vi "Remove Task.vi"(7 "Project Store in":refnum<class "Project Store.lvclass">, 8 "error in (no error)":errorcluster, 11 "ID":string) -> (0 "error out":errorcluster, 3 "found?":bool, 5 "Project Store out":refnum<class "Project Store.lvclass">)   [LabVIEW 2024, in "Project Store.lvclass"]
doc: "Removes the task with the given ID from the in-memory model. found? is FALSE when no task has that ID. Nothing is written to disk until Write to Data Source.\n\nGenerated by: Claude"
uses:
  Project Store.lvclass
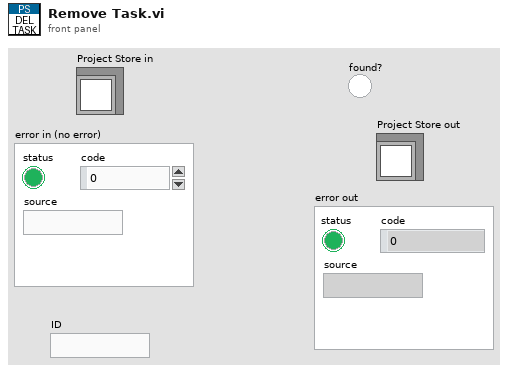
[diagram p1: front panel]
types:
  T1 = typedef "Task List.ctl" = T2[]
  T2 = typedef "Task.ctl" = cluster{"ID":string, "Project ID":string, "Name":string, "Active":bool, "Sort Order":i32}
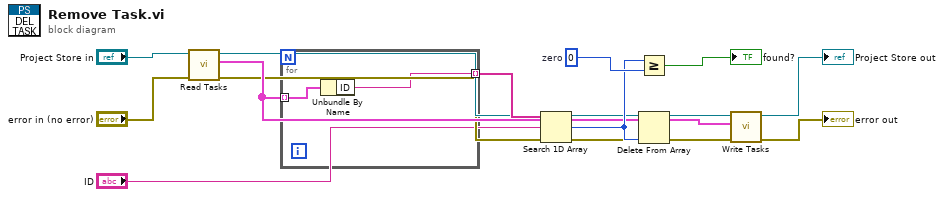
[diagram p0: block diagram]
diagram:
  w9 = 0  # zero
  n1 = call-dynamic "Read Tasks.vi"("error in (no error)"="error in (no error)", "Project Store in"="Project Store in") -> ("error out"=w4:errorcluster, "Task List"=w6:T1, "Project Store out"=w5:refnum<class "Project Store.lvclass">)  [unwired: 7 in]
  n2 = for {
    tunnel: w6 -> [w14] mode=indexing
    tunnel: [w15] -> w7 mode=indexing
    n3 = Unbundle By Name(w14) -> ("ID"=w15:string)
  }
  n4 = Search 1D Array(1D array=w7, element="ID") -> (index of element=w8:i32)  [unwired: 1 in]
  n5 = Greater Or Equal?(x=w8, y=w9) -> (x >= y?=→"found?":bool)
  n6 = Delete From Array(array=w6, index=w8) -> (array with subset deleted=w11:T1)  [unwired: 1 in, 1 out]
  n7 = call-dynamic "Write Tasks.vi"("error in (no error)"=w4, "Task List"=w11, "Project Store in"=w5) -> ("error out"=→"error out":errorcluster, "Project Store out"=→"Project Store out":refnum<class "Project Store.lvclass">)  [unwired: 7 in]
